vi "close.vi"(8 "error in":errorcluster, 11 "SystemLin Tag Module runtime in":refnum<class "SystemLink runtime.lvclass">) -> (0 "error out":errorcluster)   [LabVIEW 2015, in "SystemLink runtime.lvclass"]
doc: "Provides an interface for terminating a module instance. While this interface performs no operations, a child should close and deallocate any open references or memory."
uses:
  SystemLink runtime.lvclass
  SystemLink runtime.lvclass/SystemLink runtime.ctl
  <vilib>/Skyline/Tag/Wrapper/Wrapper_class/Close Tag (Single).vi
  <vilib>/Skyline/Configuration/Configuration_class/NI Skyline Configuration.lvclass
  <vilib>/Skyline/Tag/Wrapper/Wrapper_class/NI Skyline Tag.lvclass
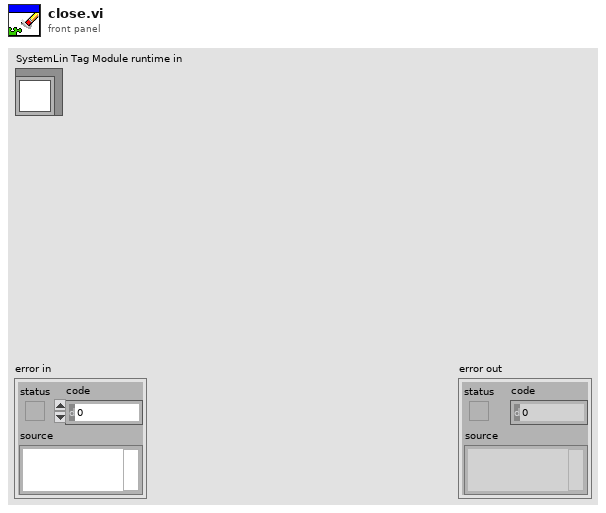
[diagram p1: front panel]
types:
  T1 = typedef "SystemLink configuration.lvclass/SysLink Mapping.ctl" = cluster{"Data Type":T2, "Tag Reference":refnum<class "NI Skyline Tag.lvclass">, "Tag Bus Index":i32, "AMQP":bool, "Skylink Index":i32}
  T2 = typedef "SystemLink configuration.lvclass/Data Tag Type.ctl" = enum16{"Double", "Single", "I32", "I16", "I8", "U64", "U32", "U16", "U8", "Boolean", "String", "Timestamp"}
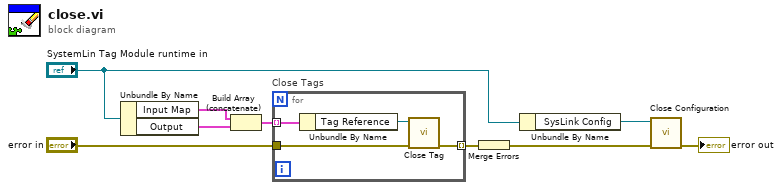
[diagram p0: block diagram]
diagram:
  n1 = Unbundle By Name("SystemLin Tag Module runtime in") -> ("Input Map"=w9:T1[], "Output"=w8:T1[])
  n2 = Build Array (concatenate)(w9, w8) -> (w7:T1[])
  n3 = for "Close Tags" {
    tunnel: w7 -> [w13] mode=indexing
    tunnel: [w11] -> w6 mode=indexing
    tunnel: "error in" -> [w10]
    n4 = Unbundle By Name(w13) -> ("Tag Reference"=w12:refnum<class "NI Skyline Tag.lvclass">)
    n5 = call-poly <vilib>:"Close Tag.vi"("error in (no error)"=w10, "tag in"=w12) -> ("error out"=w11:errorcluster)  [unwired: 9 in]
  }
  n6 = Merge Errors(w6) -> (w5:errorcluster)
  n7 = Unbundle By Name("SystemLin Tag Module runtime in") -> ("SysLink Config"=w1:refnum<class "NI Skyline Configuration.lvclass">)
  n8 = call-dynamic "Close Configuration.vi"("error in (no error)"=w5, "configuration in"=w1) -> ("error out"=→"error out":errorcluster)  [unwired: 9 in]
